vi "test tools call schema shapes.vi"(8 "error in (no error)":errorcluster) -> (0 "error out":errorcluster, 3 "body":string)   [LabVIEW 2020, in "MCP Server tests.lvlib"]
doc: "tools/call must convert each argument into the data type of its control. fake_tool_schema_shapes returns its inputs unchanged, so its answer shows how they arrived: an ISO 8601 timestamp, a cluster with an inner cluster (count, start timestamp) and an array of clusters, an array of variants, a 2D array of I32 and an enum given by its item name. Timestamps come back as ISO 8601 UTC strings and the enum as its item name. A second call sends a 3D array to fake_tool_array_shapes. The requests are sent with the LabVIEW HTTP Client directly."
uses:
  MCP Server tests.lvlib
  18665324-f37d-417a-9433-5fb41375edcb.vi
  a0c231eb-02ab-41b4-9865-a2f69dd15acf.vi
  deb57cbd-4220-48eb-9916-7e9849c0fc9b.vi
  <vilib>/JDP Science/JSONtext/Next JSON Value.vi
  <vilib>/JDP Science/JSONtext/String Subset.vi
  <vilib>/JDP Science/JSONtext/Parsing/Advance past next JSON Value (inlined COPY).vi
  <vilib>/JDP Science/JSONtext/Parsing/Advance past whitespace.vi
  <vilib>/JDP Science/JSONtext/Parsing/Advance past String.vi
  <vilib>/JDP Science/JSONtext/Parsing/Advance past Number.vi
  <vilib>/JDP Science/JSONtext/Parsing/Advance past Line Ending.vi
  <vilib>/JDP Science/JSONtext/Parsing/Parse Full Path or Item Name.vi
  <vilib>/JDP Science/JSONtext/Parsing/Advance past Array.vi
  <vilib>/JDP Science/JSONtext/Parsing/Advance past Object.vi
  <vilib>/JDP Science/JSONtext/support/Error Cluster From Code.vi
  <vilib>/JDP Science/JSONtext/Offset/Find Item Locations by Path.vi
  <vilib>/JDP Science/JSONtext/JSON text to Variant.vi
  <vilib>/JDP Science/JSONtext/LVClass Serializer/JSONtext LVClass Serializer.lvclass
  <vilib>/addons/_JKI Toolkits/Caraya/classes/Test/Test.lvclass
  <vilib>/JDP Science/JSONtext/JSONtext.lvlib
  <vilib>/addons/_JKI Toolkits/Caraya/classes/Assert/Assert.lvclass
panel:
  out "lookup error":errorcluster
  out "body 3D array":string
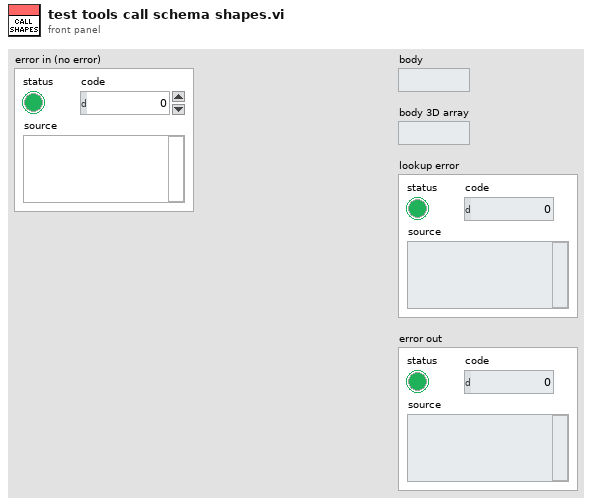
[diagram p1: front panel]
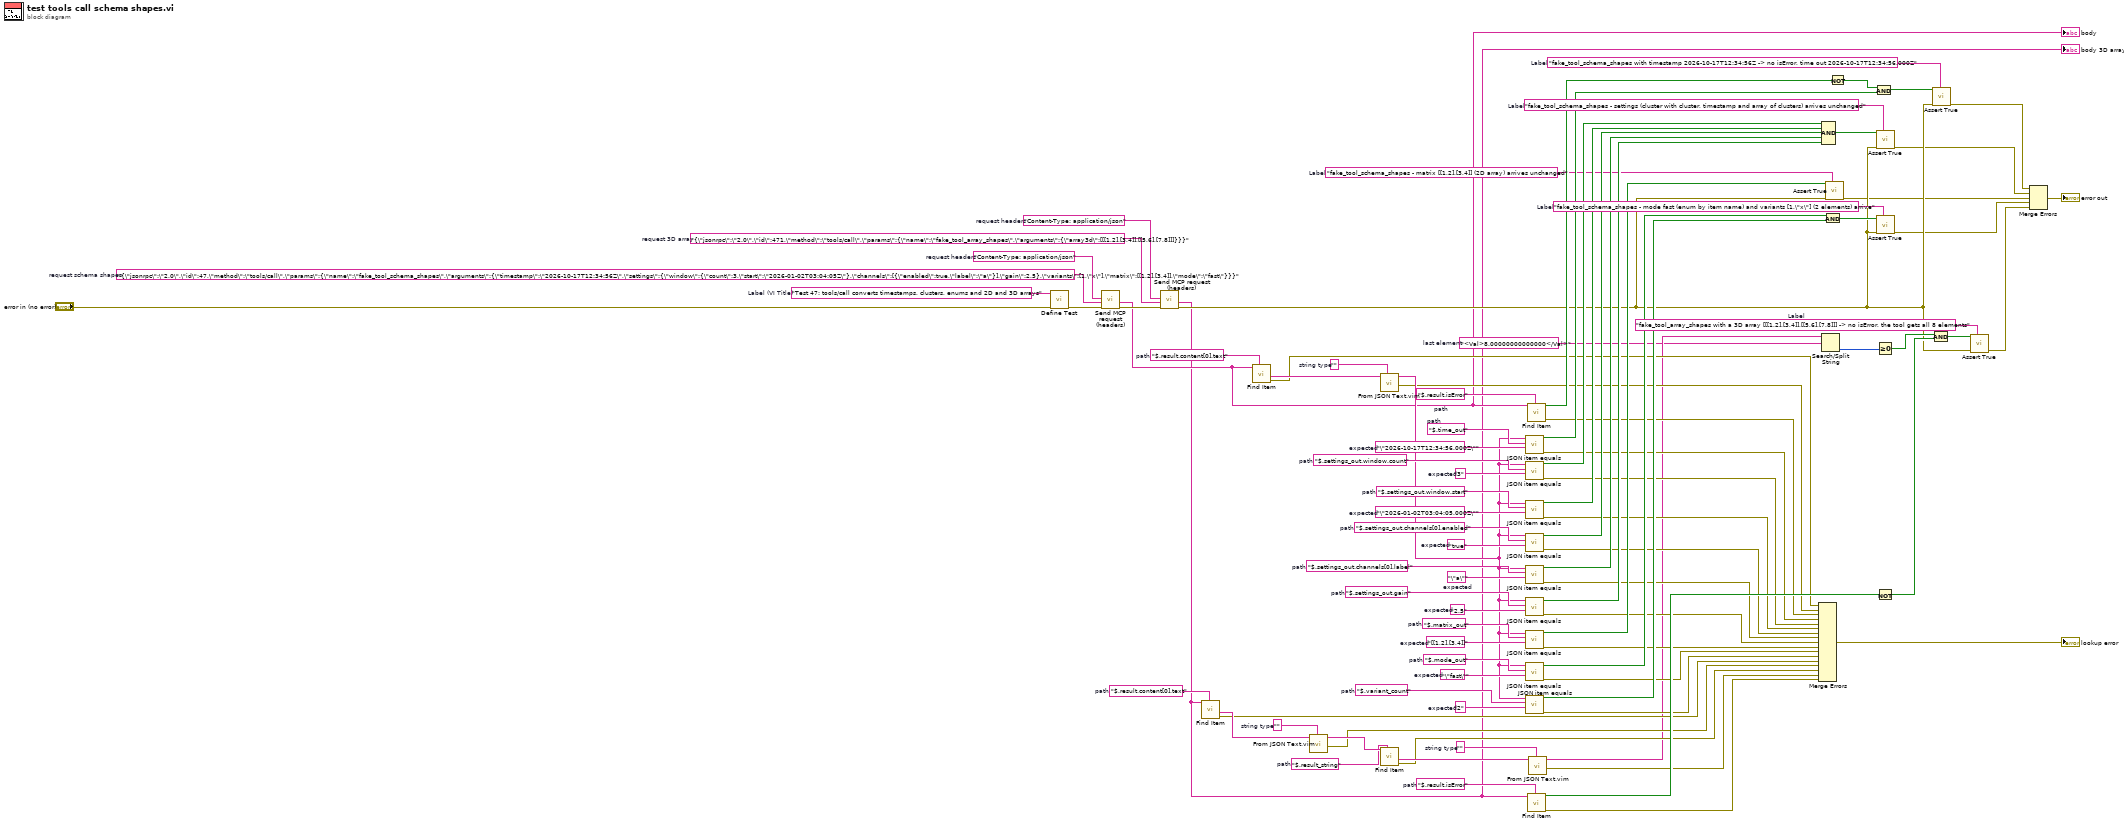
[diagram p0: block diagram]
diagram:
  w85 = "Content-Type: application/json"  # request headers
  w90 = "Content-Type: application/json"  # request headers
  w10 = "fake_tool_array_shapes with a 3D array [[[1,2],[3,4]],[[5,6],[7,8]]] -> no isError, the tool gets all 8 elements"  # Label
  w35 = "fake_tool_schema_shapes - mode fast (enum by item name) and variants [1,\"x\"] (2 elements) arrive"  # Label
  w45 = "fake_tool_schema_shapes - matrix [[1,2],[3,4]] (2D array) arrives unchanged"  # Label
  w37 = "fake_tool_schema_shapes - settings (cluster with cluster, timestamp and array of clusters) arrives unchanged"  # Label
  w39 = "fake_tool_schema_shapes with timestamp 2026-10-17T12:34:56Z -> no isError, time out 2026-10-17T12:34:56.000Z"  # Label
  w78 = "$.result.isError"  # path
  w16 = "<Val>8.00000000000000</Val>"  # last element
  w41 = ""  # string type
  w54 = "$.result_string"  # path
  w76 = ""  # string type
  w79 = "$.result.content[0].text"  # path
  w56 = "2"  # expected
  w57 = "$.variant_count"  # path
  w59 = "\"fast\""  # expected
  w60 = "$.mode_out"  # path
  w61 = "[[1,2],[3,4]]"  # expected
  w62 = "$.matrix_out"  # path
  w63 = "2.5"  # expected
  w64 = "$.settings_out.gain"  # path
  w65 = "\"a\""  # expected
  w66 = "$.settings_out.channels[0].label"  # path
  w67 = "true"  # expected
  w68 = "$.settings_out.channels[0].enabled"  # path
  w69 = "\"2026-01-02T03:04:05.000Z\""  # expected
  w70 = "$.settings_out.window.start"  # path
  w71 = "3"  # expected
  w72 = "$.settings_out.window.count"  # path
  w73 = "\"2026-10-17T12:34:56.000Z\""  # expected
  w74 = "$.time_out"  # path
  w86 = "$.result.isError"  # path
  w81 = ""  # string type
  w87 = "$.result.content[0].text"  # path
  w84 = "{\"jsonrpc\":\"2.0\",\"id\":471,\"method\":\"tools/call\",\"params\":{\"name\":\"fake_tool_array_shapes\",\"arguments\":{\"array3d\":[[[1,2],[3,4]],[[5,6],[7,8]]]}}}"  # request 3D array
  w89 = "{\"jsonrpc\":\"2.0\",\"id\":47,\"method\":\"tools/call\",\"params\":{\"name\":\"fake_tool_schema_shapes\",\"arguments\":{\"timestamp\":\"2026-10-17T12:34:56Z\",\"settings\":{\"window\":{\"count\":3,\"start\":\"2026-01-02T03:04:05Z\"},\"channels\":[{\"enabled\":true,\"label\":\"a\"}],\"gain\":2.5},\"variants\":[1,\"x\"],\"matrix\":[[1,2],[3,4]],\"mode\":\"fast\"}}}"  # request schema shapes
  w92 = "Test 47: tools/call converts timestamps, clusters, enums and 2D and 3D arrays"  # Label (VI Title)
  n1 = call <vilib>:"Define Test.vi"("error in (no error)"="error in (no error)", "Label (VI Title)"=w92) -> ("error out"=w88:errorcluster)  [unwired: 8 in, 1 out]
  n2 = call "Send MCP request (headers).vi"("error in (no error)"=w88, "request"=w89, "request headers"=w90) -> ("error out"=w83:errorcluster, "response"=w4:string)  [unwired: 5 in, 2 out]
  "body" <- w4
  n3 = call "Send MCP request (headers).vi"("error in (no error)"=w83, "request"=w84, "request headers"=w85) -> ("error out"=w11:errorcluster, "response"=w3:string)  [unwired: 5 in, 2 out]
  "body 3D array" <- w3
  n4 = call <vilib>:"Find Item.vi"("$Path or Item Name"=w79, "JSON"=w3) -> ("error out"=w22:errorcluster, "<JSON>"=w77:string)  [unwired: 6 in, 2 out]
  n5 = call <vilib>:"Find Item.vi"("$Path or Item Name"=w87, "JSON"=w4) -> ("error out"=w34:errorcluster, "<JSON>"=w82:string)  [unwired: 6 in, 2 out]
  n6 = call "From JSON Text.vim"("Data Type and Default Value"=w76, "JSON"=w77) -> ("error out"=w21:errorcluster, "Data out"=w55:string)  [unwired: 8 in]
  n7 = call "From JSON Text.vim"("Data Type and Default Value"=w81, "JSON"=w82) -> ("error out"=w33:errorcluster, "Data out"=w58:string)  [unwired: 8 in]
  n8 = call <vilib>:"Find Item.vi"("$Path or Item Name"=w54, "JSON"=w55) -> ("error out"=w20:errorcluster, "<JSON>"=w42:string)  [unwired: 6 in, 2 out]
  n9 = call "JSON item equals.vi"("expected"=w73, "path"=w74, "JSON"=w58) -> ("error out"=w31:errorcluster, "equal?"=w52:bool)  [unwired: 6 in, 1 out]
  n10 = call "JSON item equals.vi"("expected"=w71, "path"=w72, "JSON"=w58) -> ("error out"=w30:errorcluster, "equal?"=w51:bool)  [unwired: 6 in, 1 out]
  n11 = call "JSON item equals.vi"("expected"=w69, "path"=w70, "JSON"=w58) -> ("error out"=w29:errorcluster, "equal?"=w50:bool)  [unwired: 6 in, 1 out]
  n12 = call "JSON item equals.vi"("expected"=w67, "path"=w68, "JSON"=w58) -> ("error out"=w28:errorcluster, "equal?"=w49:bool)  [unwired: 6 in, 1 out]
  n13 = call "JSON item equals.vi"("expected"=w65, "path"=w66, "JSON"=w58) -> ("error out"=w27:errorcluster, "equal?"=w48:bool)  [unwired: 6 in, 1 out]
  n14 = call "JSON item equals.vi"("expected"=w63, "path"=w64, "JSON"=w58) -> ("error out"=w26:errorcluster, "equal?"=w47:bool)  [unwired: 6 in, 1 out]
  n15 = call "JSON item equals.vi"("expected"=w61, "path"=w62, "JSON"=w58) -> ("error out"=w25:errorcluster, "equal?"=w46:bool)  [unwired: 6 in, 1 out]
  n16 = call "JSON item equals.vi"("expected"=w59, "path"=w60, "JSON"=w58) -> ("error out"=w24:errorcluster, "equal?"=w44:bool)  [unwired: 6 in, 1 out]
  n17 = call "JSON item equals.vi"("expected"=w56, "path"=w57, "JSON"=w58) -> ("error out"=w23:errorcluster, "equal?"=w43:bool)  [unwired: 6 in, 1 out]
  n18 = call <vilib>:"Find Item.vi"("$Path or Item Name"=w86, "JSON"=w4) -> ("error out"=w32:errorcluster, "Found"=w80:bool)  [unwired: 6 in, 2 out]
  n19 = call <vilib>:"Find Item.vi"("$Path or Item Name"=w78, "JSON"=w3) -> ("error out"=w18:errorcluster, "Found"=w75:bool)  [unwired: 6 in, 2 out]
  n20 = call "From JSON Text.vim"("Data Type and Default Value"=w41, "JSON"=w42) -> ("error out"=w19:errorcluster, "Data out"=w17:string)  [unwired: 8 in]
  n21 = Merge Errors(w34, w33, w32, w31, w30, w29, w28, w27, w26, w25, w24, w23, w22, w21, w20, w19, w18) -> (→"lookup error":errorcluster)
  n22 = Compound Arithmetic op=AND(w51, w50, w49, w48, w47) -> (w38:bool)
  n23 = Search/Split String(string=w17, search string/char (-)=w16) -> (offset of match=w15:i32)  [unwired: 1 in, 2 out]
  n24 = call <vilib>:"Assert True.vi"("Label"=w45, "error in (no error)"=w11, "True?"=w46) -> ("error out"=w7:errorcluster)  [unwired: 7 in, 1 out]
  n25 = Compound Arithmetic op=AND(w44, w43) -> (w36:bool)
  n26 = Not(x=w80) -> (.not. x?=w53:bool)
  n27 = call <vilib>:"Assert True.vi"("Label"=w37, "error in (no error)"=w11, "True?"=w38) -> ("error out"=w8:errorcluster)  [unwired: 7 in, 1 out]
  n28 = call <vilib>:"Assert True.vi"("Label"=w35, "error in (no error)"=w11, "True?"=w36) -> ("error out"=w6:errorcluster)  [unwired: 7 in, 1 out]
  n29 = Greater Or Equal To 0?(x=w15) -> (x >= 0?=w14:bool)
  n30 = Not(x=w75) -> (.not. x?=w13:bool)
  n31 = Compound Arithmetic op=AND(w53, w52) -> (w40:bool)
  n32 = call <vilib>:"Assert True.vi"("Label"=w39, "error in (no error)"=w11, "True?"=w40) -> ("error out"=w9:errorcluster)  [unwired: 7 in, 1 out]
  n33 = Compound Arithmetic op=AND(w14, w13) -> (w12:bool)
  n34 = call <vilib>:"Assert True.vi"("Label"=w10, "error in (no error)"=w11, "True?"=w12) -> ("error out"=w5:errorcluster)  [unwired: 7 in, 1 out]
  n35 = Merge Errors(w9, w8, w7, w6, w5) -> (→"error out":errorcluster)
